vi "Write to DB Post-Assembly.vi"(8 "error in (no error)":errorcluster, 10 "Stack names":T1, 11 "Database Entry in":refnum<class "Database Entry.lvclass">) -> (0 "error out":errorcluster, 3 "Database Entry out":refnum<class "Database Entry.lvclass">)   [LabVIEW 2021, in "Database Entry.lvclass"]
uses:
  Database Entry.lvclass
  <vilib>/Utility/file.llb/Read Delimited Spreadsheet (string).vi
  <vilib>/Utility/file.llb/Write Delimited Spreadsheet (string).vi
panel:
  out "error out py":errorcluster
  out "String Out":string="Upload Success"
  out "Data cluster":T2={"module or proto"="proto", "stack name"="some", "timeend"="1:23:45.244", "Comments"=""}
  in  "error in (no error) py":errorcluster
  # "Debug instructions\n#### The order of values in db_data_cols must match the order of values in Data cluster in Stack.lvclass: Get stack data.vi \n#### The variable names below correspond to postgres col name. LV does not neet to match the col numes but just the values. \n#### Right-click on the Data cluster on the front panel and click on 'reorder controls' to verify the order is correct in the code. \n#### The physical position of the fields is different from the actual position.\n\nIn Main VIs/python_db/postgres_tools.py, see functions 'assembly_data' and 'assembly_data_as_list'."
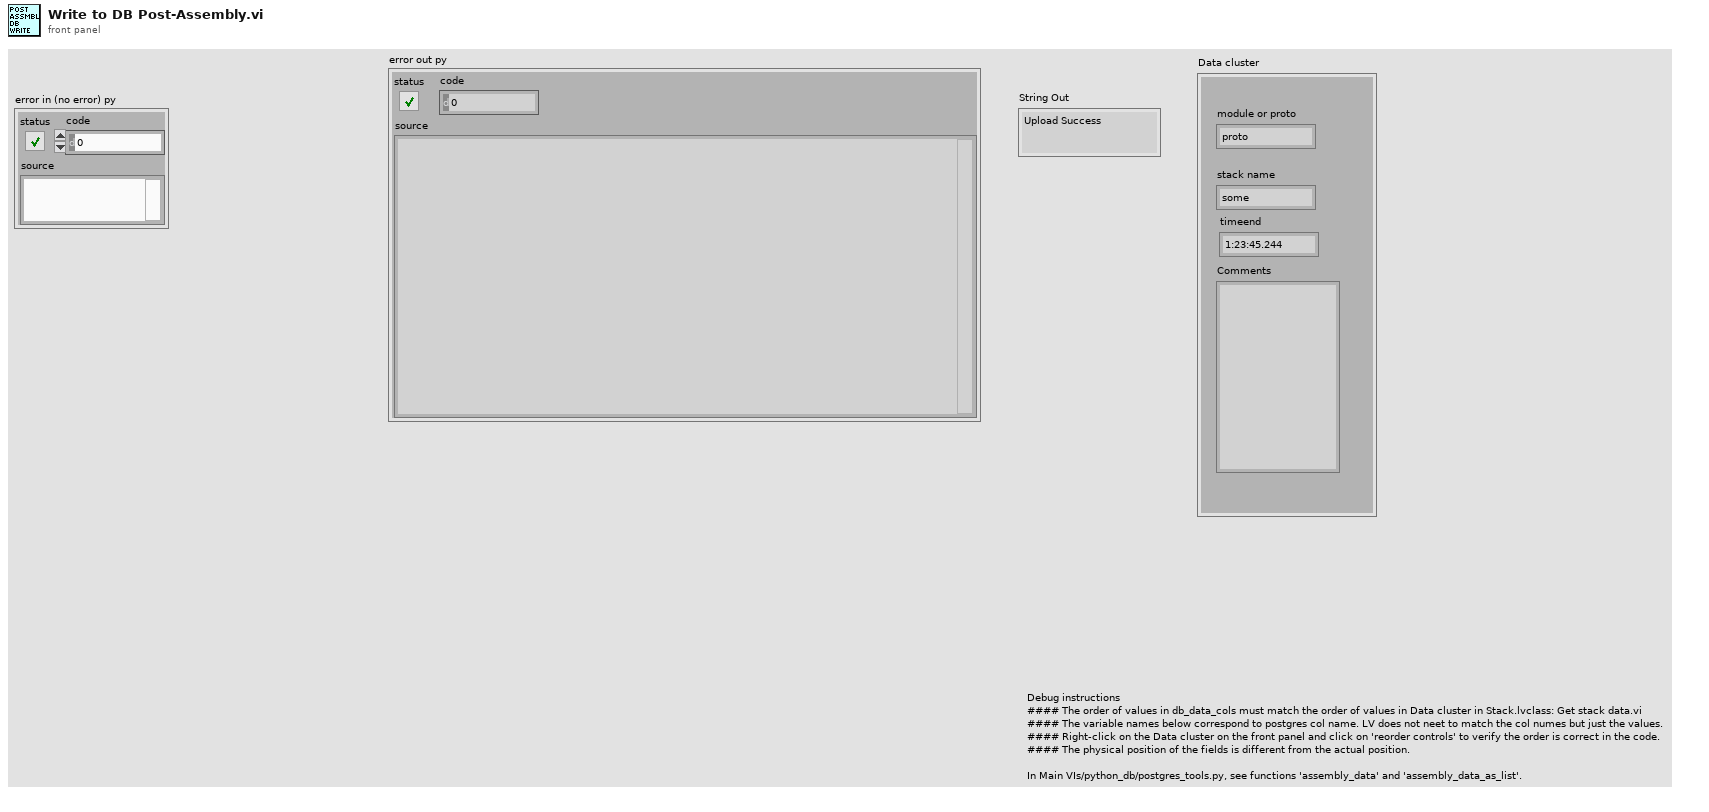
[diagram p1: front panel]
types:
  T1 = cluster{"(1) Tray 1 Pos 1":string, "(2) Tray 1 Pos 2":string, "(3) Tray 2 Pos 1":string, "(4) Tray 2 Pos 2":string}
  T2 = cluster{"module or proto":string, "stack name":string, "timeend":string, "Comments":string}
  T3 = typedef "File Paths.ctl" = cluster{"Glue Pattern Folder":path, "Carrier Tray Folder":path, "Pick Up Tool Fixture Folder":path, "Components Folder":path, "Bellows Tool Offset.txt":path, "Pick Up Tool Offset.txt":path, "Dispense Tip Offset.txt":path, "Log Files":path, "Gantry Assembly Map.txt":path, "Syringe and offset map.txt":path, "Controllers Folder":path, "Local dbase config":path}
  T4 = cluster{"(1) Tray 1 Pos 1":cluster{"Stack name":string, "Post-assembly comments":string}, "(2) Tray 1 Pos 2":cluster{"Stack name":string, "Post-assembly comments":string}, "(3) Tray 2 Pos 1":cluster{"Stack name":string, "Post-assembly comments":string}, "(4) Tray 2 Pos 2":cluster{"Stack name":string, "Post-assembly comments":string}}
  T5 = cluster{"Stack name":string, "Post-assembly comments":string}[]
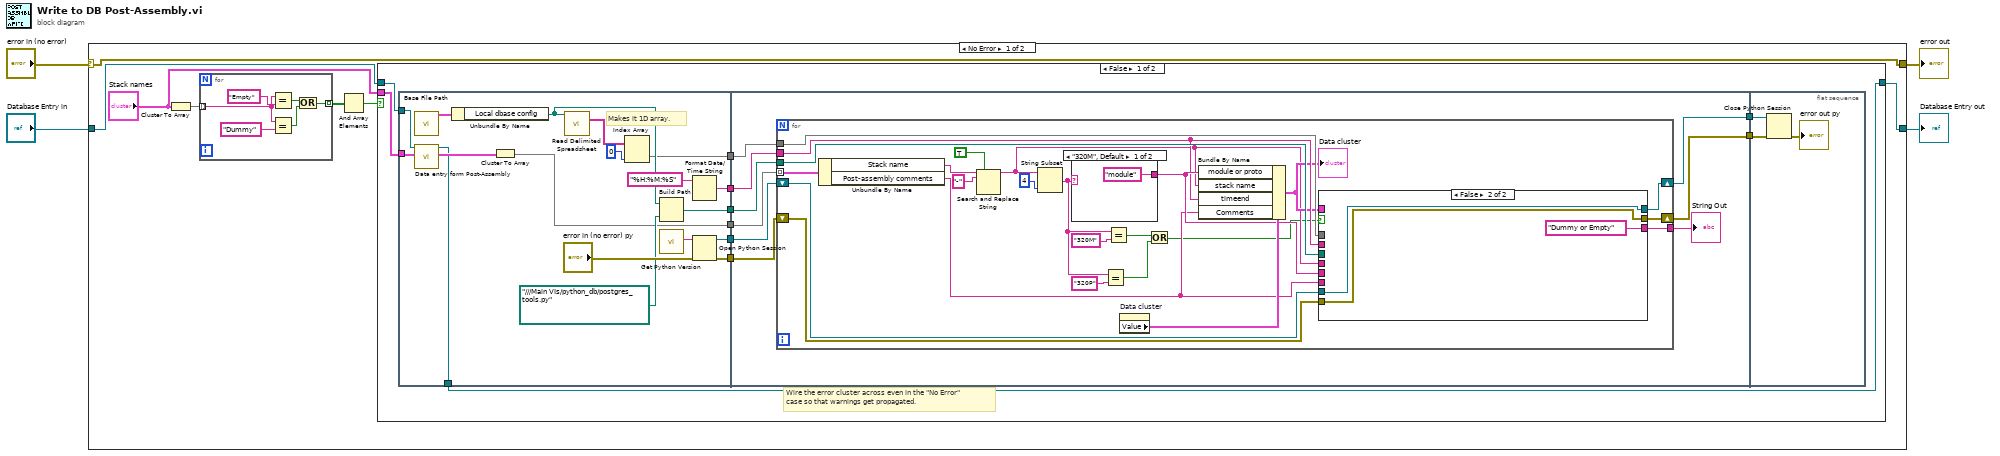
[diagram p0: block diagram]
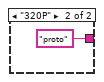
[diagram p2: hidden frame]
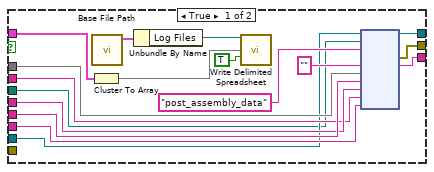
[diagram p3: hidden frame]
diagram:
  n1 = case shown="No Error" "error in (no error)" {
    selector: "error in (no error)" -> [w5 w106]
    tunnel: "Database Entry in" -> [w7 w107]
    tunnel: [w6 w107] -> w2
    tunnel: [w5 w106] -> w1
    frame No Error {
      n2 = Cluster To Array(cluster="Stack names") -> (array=w11:string[])
      n3 = for {
        tunnel: w11 -> [w103] mode=indexing
        tunnel: [w100] -> w10 mode=indexing
        n4 = Equal?(x=w103, y="Empty") -> (x = y?=w102:bool)
        n5 = Equal?(x=w103, y="Dummy") -> (x = y?=w101:bool)
        n6 = Or(x=w102, y=w101) -> (x .or. y?=w100:bool)
      }
      n7 = And Array Elements(Boolean array=w10) -> (logical AND=w9:bool)
      n8 = case shown="False" w9 {
        tunnel: "Stack names" -> [w14 _]
        tunnel: w7 -> [w13 w99]
        tunnel: [w12 w99] -> w6
        frame False {
          # "Wire the error cluster across even in the \"No Error\"\ncase so that warnings get propagated."
          n9 = flat-sequence {
            tunnel: [w39] -> w22
            tunnel: [w40] -> w21
            tunnel: [w36] -> w20
            tunnel: [w32] -> w19
            tunnel: [w29] -> w18
            tunnel: [w27] -> w17
            tunnel: w14 -> [w25]
            tunnel: w13 -> [w24]
            tunnel: [w23] -> w12
            tunnel: [w48] -> w16
            tunnel: [w47] -> w15
            tunnel: w22 -> [w49]
            tunnel: w21 -> [w46]
            tunnel: w20 -> [w45]
            tunnel: w19 -> [w44]
            tunnel: w18 -> [w42]
            tunnel: w17 -> [w41]
            tunnel: w16 -> [w97]
            tunnel: w15 -> [w98]
            frame #0 {
              # "Makes it 1D array."
              n10 = call "Base File Path.vi"() -> ("Paths Out"=w37:T3)  [unwired: 11 in]
              n11 = call "Data entry form Post-Assembly.vi"("Stack names"=w25, "Database Entry in"=w24) -> ("Post-Assembly Comments Out"=w26:T4, "Database Entry out"=w23:refnum<class "Database Entry.lvclass">)  [unwired: 7 in, 1 out]
              n12 = Unbundle By Name(w37) -> ("Local dbase config"=w35:path)
              n13 = Cluster To Array(cluster=w26) -> (array=w29:T5)
              n14 = call-poly <vilib>:"Read Delimited Spreadsheet.vi"("file path (dialog if empty)"=w35) -> ("all rows"=w34:string[][])  [unwired: 9 in, 5 out]
              n15 = Index Array(array=w34, index (col)=0 ("disabled index (col)")) -> (element=w32:string[])  [unwired: 1 in]
              n16 = Build Path(base path=w35, name or relative path=path "../../../Main VIs/python_db/postgres_tools.py" ("module path")) -> (appended path=w36:path)
              n17 = call "Get Python Version.vi"() -> ("Python Version"=w30:string)  [unwired: 10 in, 1 out]
              n18 = Format Date/Time String(time format string (%c)="%H:%M:%S") -> (date/time string=w27:string)  [unwired: 2 in]
              n19 = Open Python Session(python version=w30, 3:"error in (no error) py") -> (session out=w40:refnum<k35>, error out=w39:errorcluster)  [unwired: 1 in]
            }
            frame #1 {
              n20 = for {
                tunnel: w45 -> [w68]
                shift-right: [w73] -> w48
                shift-left: w49 -> [w67]
                shift-right: [w72] -> w47
                shift-left: w46 -> [w69]
                tunnel: [w71] -> w43
                tunnel: w44 -> [w70]
                tunnel: w42 -> [w66] mode=indexing
                tunnel: w41 -> [w62]
                n21 = Unbundle By Name(w66) -> ("Stack name"=w58:string, "Post-assembly comments"=w61:string)
                n22 = Search and Replace String(replace all?=TRUE ("replace all? (F)"), input string=w58, search string="-") -> (result string=w59:string)  [unwired: 5 in, 3 out]
                n23 = String Subset(string=w59, length (rest)=4 ("length (rest)")) -> (substring=w51:string)  [unwired: 1 in]
                n24 = case shown="\"320M\", Default" w51 {
                  tunnel: ["module" "proto"] -> w63
                  frame "320M", Default {
                  }
                  frame "320P" {
                  }
                }
                n25 = Equal?(x=w51, y="320P") -> (x = y?=w52:bool)
                n26 = Equal?(x=w51, y="320M") -> (x = y?=w53:bool)
                n27 = property on="Data cluster" class="Clust (strict)"() -> ("Value"=w65:T2)  [unwired: 2 in, 2 out]
                n28 = Or(x=w53, y=w52) -> (x .or. y?=w50:bool)
                n29 = Bundle By Name(cluster=w65, "module or proto"=w63, "stack name"=w59, "timeend"=w62, "Comments"=w61) -> (w60:T2)
                "Data cluster" <- w60
                n30 = case shown="False" w50 {
                  tunnel: [w92 w95] -> w73
                  tunnel: [w91 w93] -> w72
                  tunnel: [w90 "Dummy or Empty"] -> w71
                  tunnel: w70 -> [w88 _]
                  tunnel: w69 -> [w77 w93]
                  tunnel: w68 -> [w76 _]
                  tunnel: w67 -> [_ w95]
                  tunnel: w63 -> [w83 _]
                  tunnel: w59 -> [w82 _]
                  tunnel: w62 -> [w81 _]
                  tunnel: w61 -> [w80 _]
                  tunnel: w60 -> [w79 _]
                  frame True {
                    n31 = Cluster To Array(cluster=w79) -> (array=w78:string[])
                    n32 = call "Base File Path.vi"() -> ("Paths Out"=w86:T3)  [unwired: 11 in]
                    n33 = Unbundle By Name(w86) -> ("Log Files"=w85:path)
                    n34 = call-poly <vilib>:"Write Delimited Spreadsheet.vi"("file path (dialog if empty)"=w85, "1D data"=w78, "append to file? (new file:F)"=TRUE) -> ()  [unwired: 11 in, 2 out]
                    n35 = node(w77, w76, "post_assembly_data" ("function name"), "", w88, w83, w82, w81, w80) -> (w91:refnum<k35>, w92:errorcluster, w90:string)  [unwired: 6 in, 2 out]
                  }
                  frame False {
                  }
                }
              }
              "String Out" <- w43
            }
            frame #2 {
              n36 = Close Python Session(session in=w98, error in=w97) -> (11:→"error out py":errorcluster)
            }
          }
        }
        frame True {
        }
      }
    }
    frame Error {
    }
  }
  "Database Entry out" <- w2
  "error out" <- w1
